vi "launch_frc_robot_project_wizard.vi"() -> ()   [LabVIEW 2023]
doc: "Opens the FRC Robot Project wizard. Create Project calls this for the FRC Robot Project template (ProjectTemplates/MetaData/FRC_TemplateMetaData.xml), the same way the Getting Started window's Templates link opens it."
uses:
  <resource>/modes/FRC/Classes/ProjectWizard/ProjectWizard.lvclass
panel:
  out "error out":errorcluster
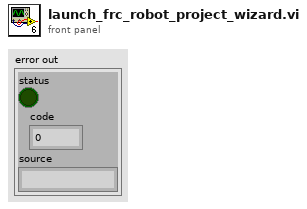
[diagram p1: front panel]
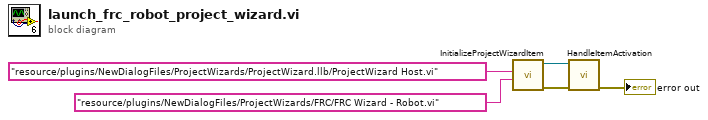
[diagram p0: block diagram]
diagram:
  n1 = call "InitializeProjectWizardItem.vi"("wizard argument"="resource/plugins/NewDialogFiles/ProjectWizards/FRC/FRC Wizard - Robot.vi", "wizard"="resource/plugins/NewDialogFiles/ProjectWizards/ProjectWizard.llb/ProjectWizard Host.vi") -> ("error out"=w3:errorcluster, "ProjectWizard out"=w2:refnum<class "ProjectWizard.lvclass">)  [unwired: 8 in]
  n2 = call <resource>:"HandleItemActivation.vi"("error in (no error)"=w3, "GettingStartedWindow.lvlib:ProjectWizard.lvclass"=w2) -> ("error out"=→"error out":errorcluster)  [unwired: 8 in, 1 out]
